vi "_test LoadUnload.vi"() -> ()   [LabVIEW 2020]
uses:
  C:/Users/Administrator/Desktop/GIT/Ballard-Arinc-429-XML-Generator/Source/Assemblies/Ballard_Parameter_ni/bin/Debug/Parameters_Arinc429_XML_Tools.dll
  Source/Assemblies/Ballard_Parameter_ni/bin/Debug/Parameters_Arinc429_XML_Tools.dll
panel:
  out "Array":T1(array[cluster])
  out "error out":errorcluster
  in  "XML path":path=path "C:/Users/Administrator/Desktop/GIT/Ballard-Arinc-429-XML-Generator/Database Examples/Parameters.xml"
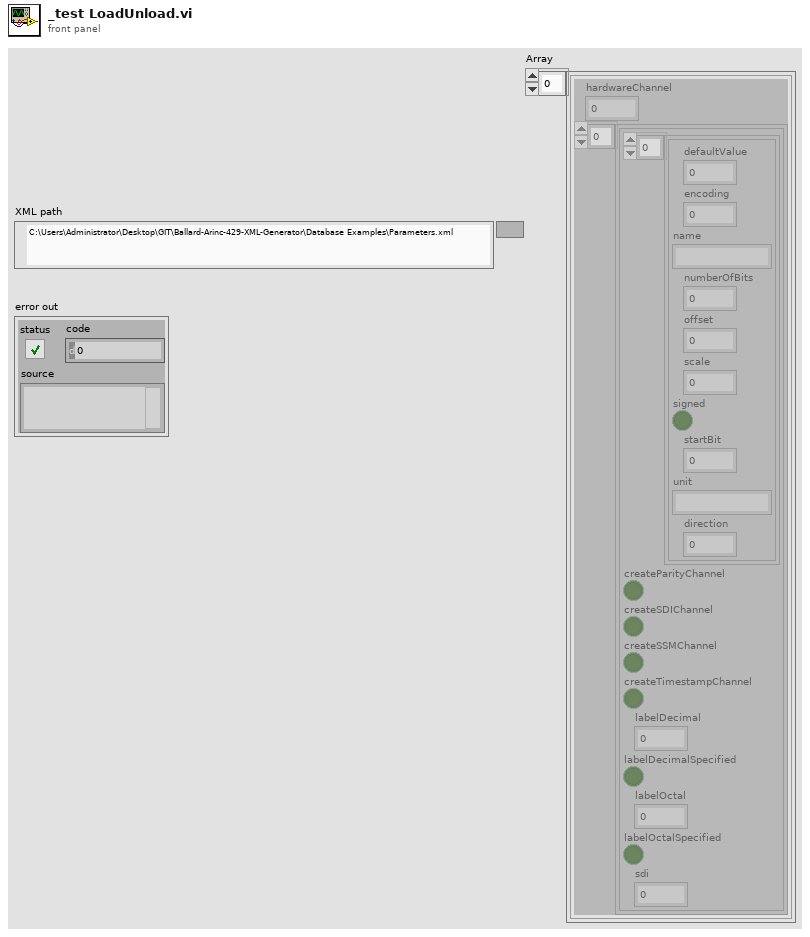
[diagram p1: front panel]
types:
  T1 = cluster{"hardwareChannel":i32, cluster{cluster{"defaultValue":dbl, "encoding":i32, "name":string, "numberOfBits":i32, "offset":dbl, "scale":dbl, "signed":bool, "startBit":i32, "unit":string, "direction":i32}[], "createParityChannel":bool, "createSDIChannel":bool, "createSSMChannel":bool, "createTimestampChannel":bool, "labelDecimal":i32, "labelDecimalSpecified":bool, "labelOctal":i32, "labelOctalSpecified":bool, "sdi":i32}[]}[]
  T2 = cluster{"defaultValue":dbl, "encoding":i32, "name":string, "numberOfBits":i32, "offset":dbl, "scale":dbl, "signed":bool, "startBit":i32, "unit":string, "direction":i32}
  T3 = cluster{cluster{"defaultValue":dbl, "encoding":i32, "name":string, "numberOfBits":i32, "offset":dbl, "scale":dbl, "signed":bool, "startBit":i32, "unit":string, "direction":i32}[], "createParityChannel":bool, "createSDIChannel":bool, "createSSMChannel":bool, "createTimestampChannel":bool, "labelDecimal":i32, "labelDecimalSpecified":bool, "labelOctal":i32, "labelOctalSpecified":bool, "sdi":i32}
  T4 = cluster{"hardwareChannel":i32, cluster{cluster{"defaultValue":dbl, "encoding":i32, "name":string, "numberOfBits":i32, "offset":dbl, "scale":dbl, "signed":bool, "startBit":i32, "unit":string, "direction":i32}[], "createParityChannel":bool, "createSDIChannel":bool, "createSSMChannel":bool, "createTimestampChannel":bool, "labelDecimal":i32, "labelDecimalSpecified":bool, "labelOctal":i32, "labelOctalSpecified":bool, "sdi":i32}[]}
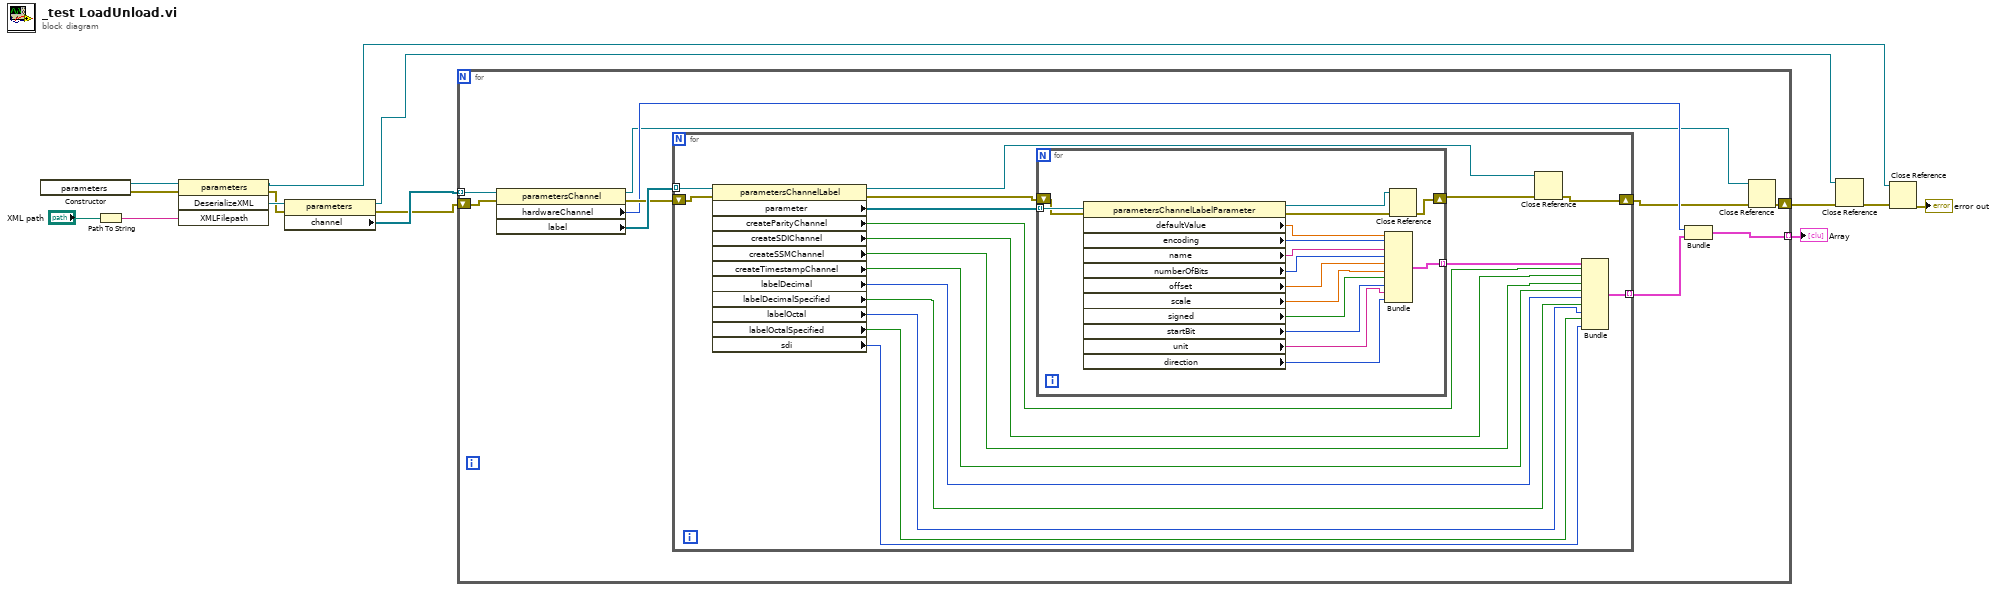
[diagram p0: block diagram]
diagram:
  n1 = constructor class="parameters"() -> (reference out=w14:refnum<k24>, error out=w13:errorcluster)  [unwired: 3 in, 1 out]
  n2 = Path To String(path="XML path") -> (string=w11:string)
  n3 = invoke class="parameters" method="DeserializeXML"(reference=w14, error in=w13, "XMLFilepath"=w11) -> (reference out=w3:refnum<k24>, error out=w9:errorcluster, "DeserializeXML"=w10:refnum<k24>)  [unwired: 1 in, 1 out]
  n4 = property class="parameters"(reference=w10, error in=w9) -> (reference out=w6:refnum<k24>, error out=w7:errorcluster, "channel"=w8:refnum<k24>[])
  n5 = for {
    tunnel: w8 -> [w24] mode=indexing
    shift-right: [w16] -> w5
    shift-left: w7 -> [w23]
    tunnel: [w15] -> w1 mode=indexing
    n6 = property class="parametersChannel"(reference=w24, error in=w23) -> (reference out=w18:refnum<k24>, error out=w21:errorcluster, "hardwareChannel"=w20:i32, "label"=w22:refnum<k24>[])
    n7 = for {
      tunnel: w22 -> [w42] mode=indexing
      shift-right: [w25] -> w17
      shift-left: w21 -> [w41]
      tunnel: [w26] -> w19 mode=indexing
      n8 = property class="parametersChannelLabel"(reference=w42, error in=w41) -> (reference out=w38:refnum<k24>, error out=w40:errorcluster, "parameter"=w39:refnum<k24>[], "createParityChannel"=w35:bool, "createSDIChannel"=w34:bool, "createSSMChannel"=w33:bool, "createTimestampChannel"=w32:bool, "labelDecimal"=w31:i32, "labelDecimalSpecified"=w30:bool, "labelOctal"=w29:i32, "labelOctalSpecified"=w28:bool, "sdi"=w27:i32)
      n9 = for {
        tunnel: w39 -> [w58] mode=indexing
        tunnel: [w47] -> w36 mode=indexing
        shift-right: [w45] -> w37
        shift-left: w40 -> [w57]
        n10 = property class="parametersChannelLabelParameter"(reference=w58, error in=w57) -> (reference out=w44:refnum<k24>, error out=w46:errorcluster, "defaultValue"=w56:dbl, "encoding"=w55:i32, "name"=w54:string, "numberOfBits"=w53:i32, "offset"=w52:dbl, "scale"=w51:dbl, "signed"=w50:bool, "startBit"=w49:i32, "unit"=w48:string, "direction"=w43:i32)
        n11 = Bundle("defaultValue"=w56, "encoding"=w55, "name"=w54, "numberOfBits"=w53, "offset"=w52, "scale"=w51, "signed"=w50, "startBit"=w49, "unit"=w48, "direction"=w43) -> (w47:T2)  [unwired: 1 in]
        n12 = Close Reference(reference=w44, error in (no error)=w46) -> (error out=w45:errorcluster)
      }
      n13 = Close Reference(reference=w38, error in (no error)=w37) -> (error out=w25:errorcluster)
      n14 = Bundle(w36, "createParityChannel"=w35, "createSDIChannel"=w34, "createSSMChannel"=w33, "createTimestampChannel"=w32, "labelDecimal"=w31, "labelDecimalSpecified"=w30, "labelOctal"=w29, "labelOctalSpecified"=w28, "sdi"=w27) -> (w26:T3)  [unwired: 1 in]
    }
    n15 = Bundle("hardwareChannel"=w20, w19) -> (w15:T4)  [unwired: 1 in]
    n16 = Close Reference(reference=w18, error in (no error)=w17) -> (error out=w16:errorcluster)
  }
  "Array" <- w1
  n17 = Close Reference(reference=w6, error in (no error)=w5) -> (error out=w4:errorcluster)
  n18 = Close Reference(reference=w3, error in (no error)=w4) -> (error out=→"error out":errorcluster)
